vi "BSD_Filename Path formation_MS.vi"(6 "BF_name":string, 8 "error in (no error)":errorcluster caption="error in", 9 "Date":string, 10 "SAVE":bool=TRUE, 11 "Filename Path":path) -> (0 "error out":errorcluster, 1 "BNAL Path":T2, 2 "LS Path":T3, 3 "BS Path":T1, 4 "FN#":string)   [LabVIEW 2018]
panel:
  out "after substring":string
  out "after substring 4":string
  out "BS_S Path":string
  out "BS_J Path":string
  out "BS_CP Path":string
  out "B_TDMS Path":string
  out "B_Folder Path":string
  out "LSE Path":string
  out "BS_T Path":string
  out "LS Signal Table Path":path
  out "LS CP Table Path":path
  out "LS Time Table Path":path
  out "Ex Con":string
  out "B_TDMS F_Name":string
  out "B_Folder name":string
  out "Pre File F_Name":string
  out "File location folder":string
  out "B Signal Table Path":path
  out "B CP Table Path":path
  out "B Time Table Path":path
  out "Filename":string
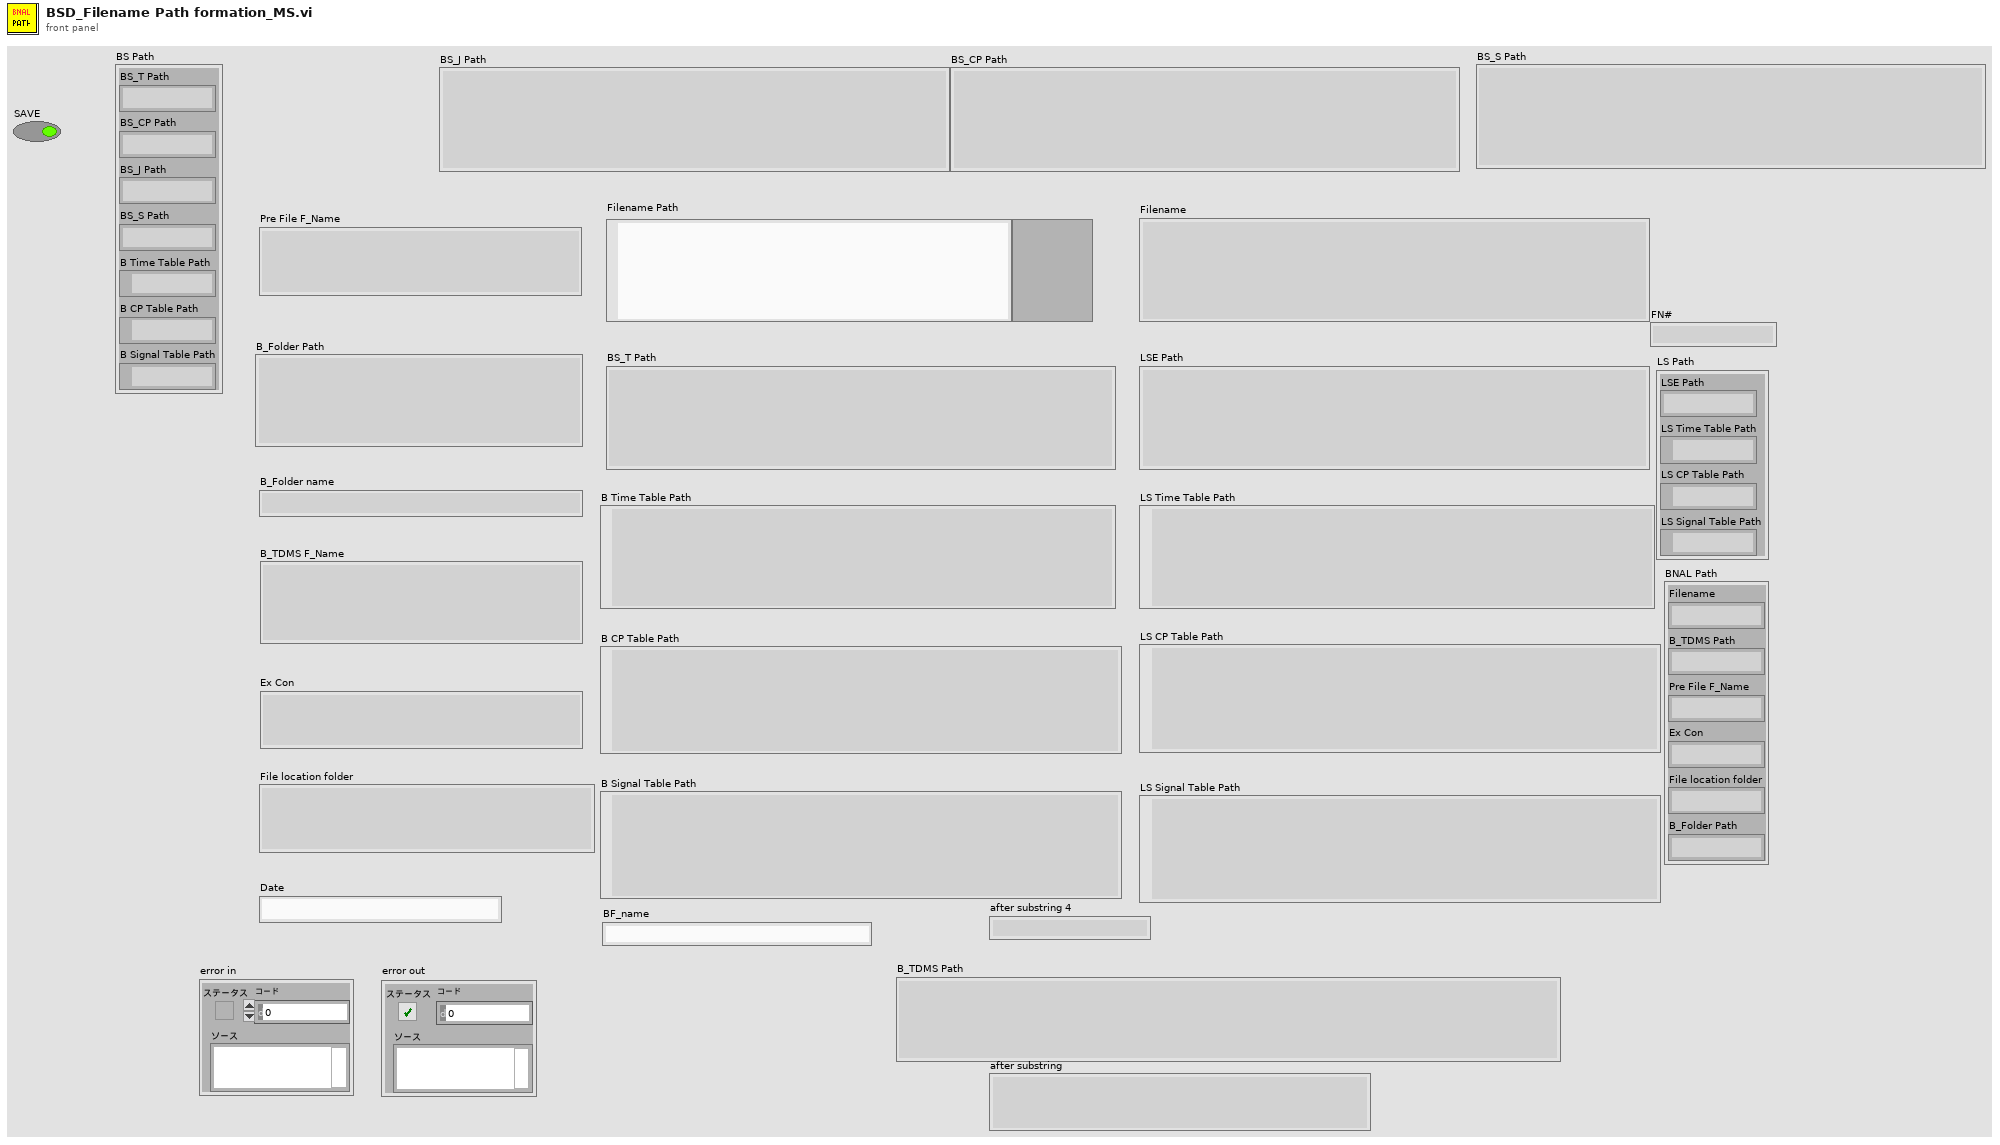
[diagram p1: front panel]
types:
  T1 = cluster{"BS_T Path":string, "BS_CP Path":string, "BS_J Path":string, "BS_S Path":string, "B Time Table Path":path, "B CP Table Path":path, "B Signal Table Path":path}
  T2 = cluster{"Filename":string, "B_TDMS Path":string, "Pre File F_Name":string, "Ex Con":string, "File location folder":string, "B_Folder Path":string}
  T3 = cluster{"LSE Path":string, "LS Time Table Path":path, "LS CP Table Path":path, "LS Signal Table Path":path}
  T4 = cluster{"name":string, string, string, string, string, string}
  T5 = cluster{string, string, string, string, path, path, path}
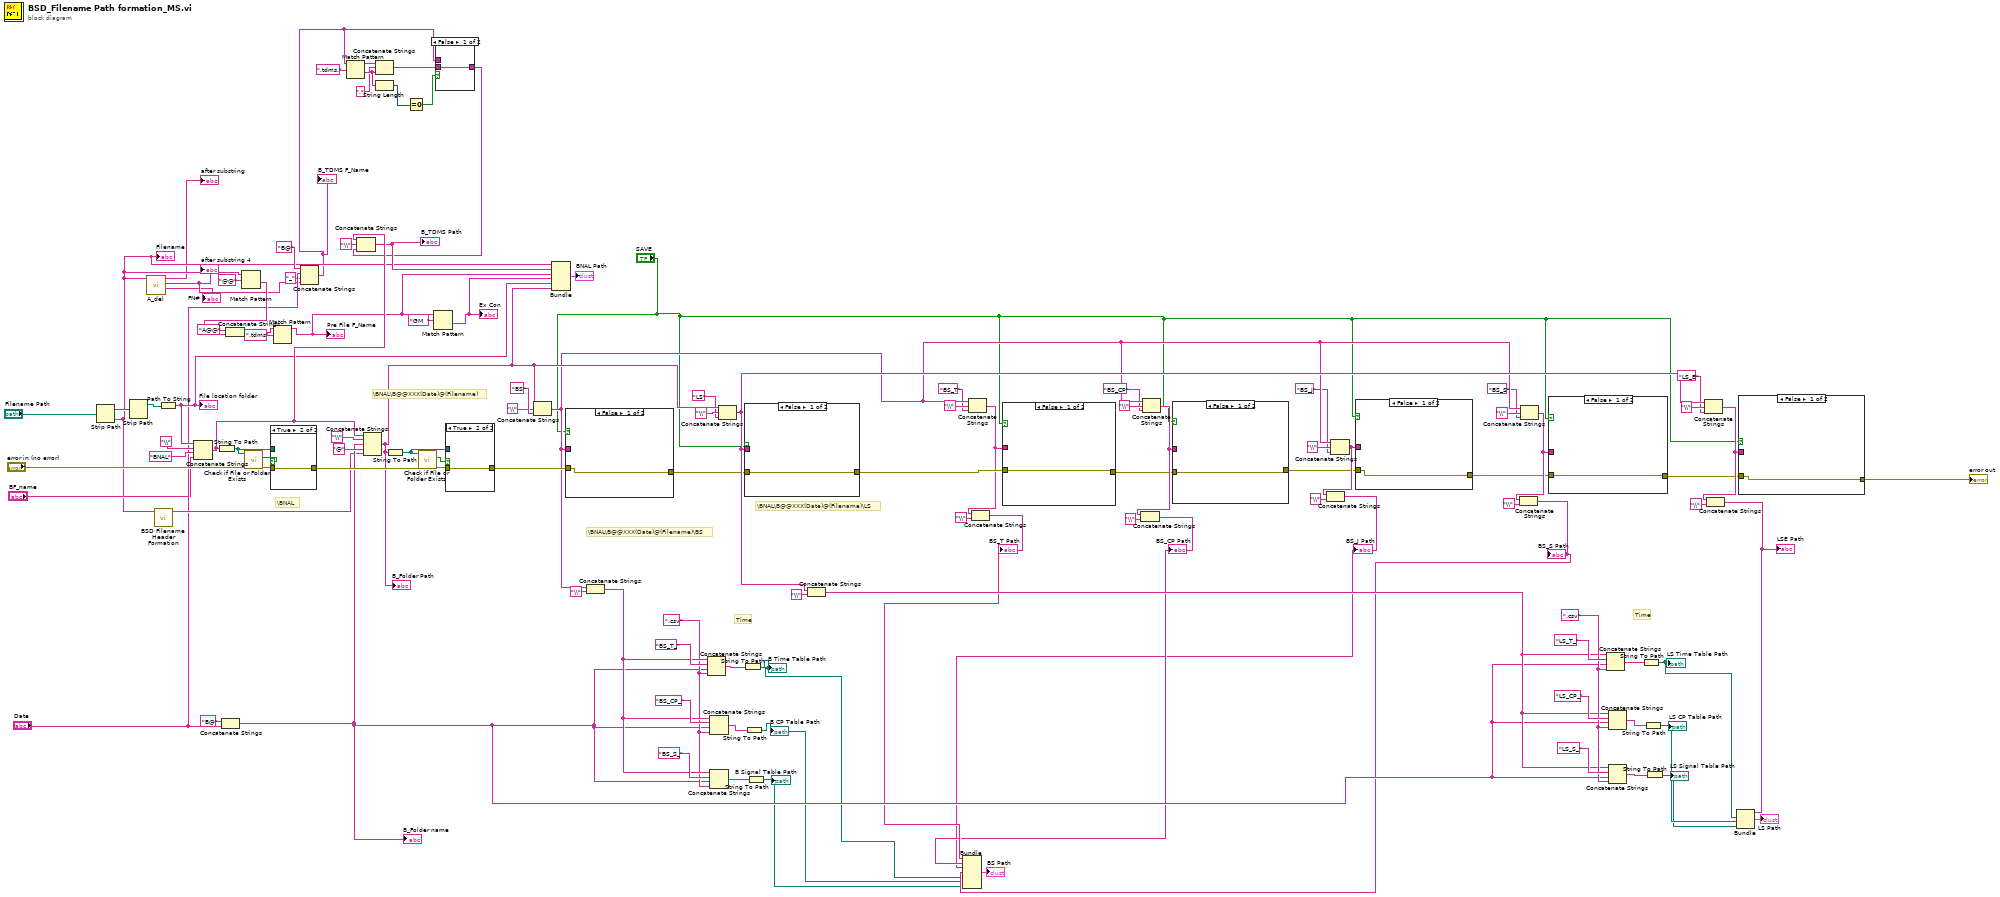
[diagram p0: block diagram]
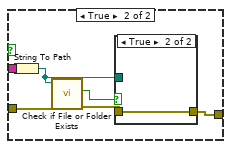
[diagram p3: hidden frame]
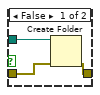
[diagram p4: hidden frame]
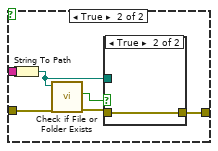
[diagram p5: hidden frame]
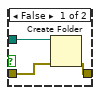
[diagram p6: hidden frame]
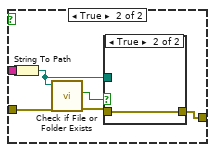
[diagram p7: hidden frame]
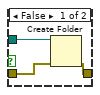
[diagram p8: hidden frame]
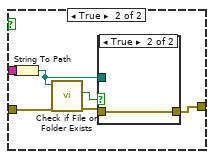
[diagram p9: hidden frame]
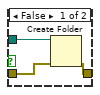
[diagram p10: hidden frame]
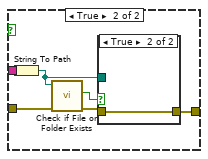
[diagram p11: hidden frame]
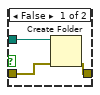
[diagram p12: hidden frame]
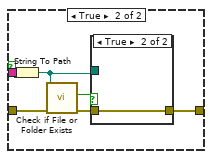
[diagram p13: hidden frame]
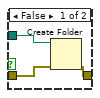
[diagram p14: hidden frame]
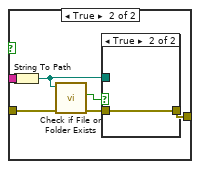
[diagram p15: hidden frame]
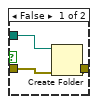
[diagram p16: hidden frame]
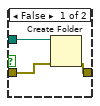
[diagram p17: hidden frame]
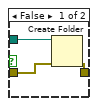
[diagram p18: hidden frame]
diagram:
  w78 = ".csv" ("文字列")
  w85 = ".csv" ("文字列")
  # "\\BNAL\\B@@XXX(Date)@(Filename)\\LS"
  # "\\BNAL\\B@@XXX(Date)@(Filename)\\BS"
  # "Time"
  # "\\BNAL\\B@@XXX(Date)@(Filename)"
  # "\\BNAL"
  # "Time"
  n1 = Strip Path(path="Filename Path") -> (stripped path=w68:path, name=w14:string)
  "Filename" <- w14
  n2 = Strip Path(path=w68) -> (stripped path=w87:path)  [unwired: 1 out]
  n3 = call "A_del.vi"("Filename"=w14) -> ("before substring 2"=→"FN#":string, "after substring 4"=w13:string, "after substring"=→"after substring":string)  [unwired: 8 in]
  "after substring 4" <- w13
  n4 = call "BSD Filename Header Formation.vi"("Pre File F_Name"=w14) -> ("Head for BNAL"=w49:string)  [unwired: 10 in]
  n5 = Path To String(path=w87) -> (string=w60:string)
  "File location folder" <- w60
  n6 = Concatenate Strings(w60, "\\" ("文字列"), "BNAL" ("文字列"), "BF_name") -> (w66:string)
  n7 = String To Path(string=w66) -> (path=w104:path)
  n8 = Concatenate Strings("B@" ("文字列"), "Date") -> (w76:string)
  "B_Folder name" <- w76
  n9 = Match Pattern(string=w14, regular expression="@@" ("正規表現")) -> (after substring=w50:string)  [unwired: 1 in, 3 out]
  n10 = Concatenate Strings("A@@" ("文字列"), w50) -> (w91:string)
  n11 = call <vilib>:"Check if File or Folder Exists.vi"("error in (no error)"="error in (no error)", "path"=w104) -> ("error out"=w102:errorcluster, "file or folder exists?"=w103:bool)  [unwired: 7 in, 1 out]
  n12 = case shown="True" w103 {
    tunnel: w104 -> [w118 _]
    tunnel: w102 -> [w117 w119]
    tunnel: [w116 w119] -> w95
    frame False {
      n13 = Create Folder(path (use dialog)=w118, error in=w117) -> (error out=w116:errorcluster)  [unwired: 1 in, 2 out]
    }
    frame True {
    }
  }
  n14 = Match Pattern(string=w91, regular expression=".tdms" ("正規表現")) -> (before substring=w63:string)  [unwired: 1 in, 3 out]
  "Pre File F_Name" <- w63
  n15 = Concatenate Strings("B@" ("文字列"), "Date", "_" ("string"), w13) -> (w2:string)
  "B_TDMS F_Name" <- w2
  n16 = Match Pattern(string=w2, regular expression=".tdms.") -> (before substring=w6:string, after substring=w5:string)  [unwired: 1 in, 2 out]
  n17 = Concatenate Strings(w66, "\\" ("文字列"), w76, "@" ("文字列"), w49) -> (w61:string)
  "B_Folder Path" <- w61
  n18 = Concatenate Strings(w6, "." ("string"), w5) -> (w3:string)
  n19 = String Length(string=w5) -> (length=w8:i32)
  n20 = String To Path(string=w61) -> (path=w98:path)
  n21 = Equal To 0?(x=w8) -> (x = 0?=w7:bool)
  n22 = call <vilib>:"Check if File or Folder Exists.vi"("error in (no error)"=w95, "path"=w98) -> ("error out"=w96:errorcluster, "file or folder exists?"=w97:bool)  [unwired: 7 in, 1 out]
  n23 = Match Pattern(string=w63, regular expression="GM  " ("正規表現")) -> (after substring=w62:string)  [unwired: 1 in, 3 out]
  "Ex Con" <- w62
  n24 = case shown="False" w7 {
    tunnel: w2 -> [_ w121]
    tunnel: [w120 w121] -> w1
    tunnel: w3 -> [w120 _]
    frame False {
    }
    frame True {
    }
  }
  n25 = Concatenate Strings(w66, "\\" ("文字列"), w1) -> (w64:string)
  "B_TDMS Path" <- w64
  n26 = case shown="True" w97 {
    tunnel: w98 -> [w124 _]
    tunnel: w96 -> [w123 w125]
    tunnel: [w122 w125] -> w94
    frame False {
      n27 = Create Folder(path (use dialog)=w124, error in=w123) -> (error out=w122:errorcluster)  [unwired: 1 in, 2 out]
    }
    frame True {
    }
  }
  n28 = Concatenate Strings(w61, "\\" ("文字列"), "BS" ("文字列")) -> (w51:string)
  n29 = Bundle("name"=w14, w64, w63, w62, w60, w61) -> (→"BNAL Path":T4)  [unwired: 1 in]
  n30 = case shown="False" "SAVE" {
    tunnel: w94 -> [w126 w132]
    tunnel: w51 -> [_ w131]
    tunnel: [w126 w127] -> w44
    frame False {
    }
    frame True {
      n31 = String To Path(string=w131) -> (path=w130:path)
      n32 = call <vilib>:"Check if File or Folder Exists.vi"("error in (no error)"=w132, "path"=w130) -> ("error out"=w128:errorcluster, "file or folder exists?"=w129:bool)  [unwired: 7 in, 1 out]
      n33 = case shown="True" w129 {
        tunnel: w130 -> [w135 _]
        tunnel: w128 -> [w134 w136]
        tunnel: [w133 w136] -> w127
        frame False {
          n34 = Create Folder(path (use dialog)=w135, error in=w134) -> (error out=w133:errorcluster)  [unwired: 1 in, 2 out]
        }
        frame True {
        }
      }
    }
  }
  n35 = Concatenate Strings(w51, "\\" ("文字列")) -> (w86:string)
  n36 = Concatenate Strings(w86, "BS_T_" ("文字列"), w76, w85) -> (w113:string)
  n37 = Concatenate Strings(w86, "BS_CP_" ("文字列"), w76, w85) -> (w112:string)
  n38 = Concatenate Strings(w86, "BS_S_" ("文字列"), w76, w85) -> (w111:string)
  n39 = Concatenate Strings(w61, "\\" ("文字列"), "LS" ("文字列")) -> (w75:string)
  n40 = String To Path(string=w113) -> (path=w54:path)
  "B Time Table Path" <- w54
  n41 = case shown="False" "SAVE" {
    tunnel: w75 -> [_ w143]
    tunnel: w44 -> [w137 w140]
    tunnel: [w137 w139] -> w43
    frame False {
    }
    frame True {
      n42 = String To Path(string=w143) -> (path=w138:path)
      n43 = call <vilib>:"Check if File or Folder Exists.vi"("error in (no error)"=w140, "path"=w138) -> ("error out"=w141:errorcluster, "file or folder exists?"=w142:bool)  [unwired: 7 in, 1 out]
      n44 = case shown="True" w142 {
        tunnel: w138 -> [w146 _]
        tunnel: w141 -> [w145 w147]
        tunnel: [w144 w147] -> w139
        frame False {
          n45 = Create Folder(path (use dialog)=w146, error in=w145) -> (error out=w144:errorcluster)  [unwired: 1 in, 2 out]
        }
        frame True {
        }
      }
    }
  }
  n46 = String To Path(string=w112) -> (path=w53:path)
  "B CP Table Path" <- w53
  n47 = String To Path(string=w111) -> (path=w52:path)
  "B Signal Table Path" <- w52
  n48 = Concatenate Strings(w75, "\\" ("文字列")) -> (w77:string)
  n49 = Concatenate Strings(w51, "\\" ("文字列"), "BS_T" ("文字列")) -> (w38:string)
  n50 = Concatenate Strings(w38, "\\" ("文字列")) -> (w58:string)
  "BS_T Path" <- w58
  n51 = case shown="False" "SAVE" {
    tunnel: w43 -> [w148 w152]
    tunnel: w38 -> [_ w150]
    tunnel: [w148 w149] -> w28
    frame False {
    }
    frame True {
      n52 = String To Path(string=w150) -> (path=w151:path)
      n53 = call <vilib>:"Check if File or Folder Exists.vi"("error in (no error)"=w152, "path"=w151) -> ("error out"=w153:errorcluster, "file or folder exists?"=w154:bool)  [unwired: 7 in, 1 out]
      n54 = case shown="True" w154 {
        tunnel: w151 -> [w157 _]
        tunnel: w153 -> [w156 w158]
        tunnel: [w155 w158] -> w149
        frame False {
          n55 = Create Folder(path (use dialog)=w157, error in=w156) -> (error out=w155:errorcluster)  [unwired: 1 in, 2 out]
        }
        frame True {
        }
      }
    }
  }
  n56 = Concatenate Strings(w51, "\\" ("文字列"), "BS_CP" ("文字列")) -> (w29:string)
  n57 = Concatenate Strings(w29, "\\" ("文字列")) -> (w57:string)
  "BS_CP Path" <- w57
  n58 = case shown="False" "SAVE" {
    tunnel: w29 -> [_ w162]
    tunnel: w28 -> [w159 w161]
    tunnel: [w159 w160] -> w24
    frame False {
    }
    frame True {
      n59 = String To Path(string=w162) -> (path=w163:path)
      n60 = call <vilib>:"Check if File or Folder Exists.vi"("error in (no error)"=w161, "path"=w163) -> ("error out"=w164:errorcluster, "file or folder exists?"=w165:bool)  [unwired: 7 in, 1 out]
      n61 = case shown="True" w165 {
        tunnel: w163 -> [w168 _]
        tunnel: w164 -> [w167 w169]
        tunnel: [w166 w169] -> w160
        frame False {
          n62 = Create Folder(path (use dialog)=w168, error in=w167) -> (error out=w166:errorcluster)  [unwired: 1 in, 2 out]
        }
        frame True {
        }
      }
    }
  }
  n63 = Concatenate Strings(w51, "\\" ("文字列"), "BS_J" ("文字列")) -> (w25:string)
  n64 = Concatenate Strings(w25, "\\" ("文字列")) -> (w56:string)
  "BS_J Path" <- w56
  n65 = case shown="False" "SAVE" {
    tunnel: w25 -> [_ w173]
    tunnel: w24 -> [w170 w172]
    tunnel: [w170 w171] -> w19
    frame False {
    }
    frame True {
      n66 = String To Path(string=w173) -> (path=w174:path)
      n67 = call <vilib>:"Check if File or Folder Exists.vi"("error in (no error)"=w172, "path"=w174) -> ("error out"=w175:errorcluster, "file or folder exists?"=w176:bool)  [unwired: 7 in, 1 out]
      n68 = case shown="True" w176 {
        tunnel: w174 -> [w179 _]
        tunnel: w175 -> [w178 w180]
        tunnel: [w177 w180] -> w171
        frame False {
          n69 = Create Folder(path (use dialog)=w179, error in=w178) -> (error out=w177:errorcluster)  [unwired: 1 in, 2 out]
        }
        frame True {
        }
      }
    }
  }
  n70 = Concatenate Strings(w51, "\\" ("文字列"), "BS_S" ("文字列")) -> (w20:string)
  n71 = Concatenate Strings(w20, "\\" ("文字列")) -> (w55:string)
  "BS_S Path" <- w55
  n72 = Bundle(w58, w57, w56, w55, w54, w53, w52) -> (→"BS Path":T5)  [unwired: 1 in]
  n73 = case shown="False" "SAVE" {
    tunnel: w20 -> [_ w184]
    tunnel: w19 -> [w181 w183]
    tunnel: [w181 w182] -> w18
    frame False {
    }
    frame True {
      n74 = String To Path(string=w184) -> (path=w185:path)
      n75 = call <vilib>:"Check if File or Folder Exists.vi"("error in (no error)"=w183, "path"=w185) -> ("error out"=w186:errorcluster, "file or folder exists?"=w187:bool)  [unwired: 7 in, 1 out]
      n76 = case shown="True" w187 {
        tunnel: w185 -> [w190 _]
        tunnel: w186 -> [w189 w191]
        tunnel: [w188 w191] -> w182
        frame False {
          n77 = Create Folder(path (use dialog)=w190, error in=w189) -> (error out=w188:errorcluster)  [unwired: 1 in, 2 out]
        }
        frame True {
        }
      }
    }
  }
  n78 = Concatenate Strings(w77, "LS_T_" ("文字列"), w76, w78) -> (w84:string)
  n79 = Concatenate Strings(w77, "LS_CP_" ("文字列"), w76, w78) -> (w83:string)
  n80 = Concatenate Strings(w77, "LS_S_" ("文字列"), w76, w78) -> (w82:string)
  n81 = String To Path(string=w84) -> (path=w71:path)
  "LS Time Table Path" <- w71
  n82 = String To Path(string=w83) -> (path=w70:path)
  "LS CP Table Path" <- w70
  n83 = String To Path(string=w82) -> (path=w69:path)
  "LS Signal Table Path" <- w69
  n84 = Concatenate Strings(w75, "\\" ("文字列"), "LS_E" ("文字列")) -> (w34:string)
  n85 = Concatenate Strings(w34, "\\" ("文字列")) -> (w72:string)
  "LSE Path" <- w72
  n86 = Bundle(w72, w71, w70, w69) -> (→"LS Path":cluster{string, path, path, path})  [unwired: 1 in]
  n87 = case shown="False" "SAVE" {
    tunnel: [w192 w198] -> w74
    tunnel: w34 -> [_ w194]
    tunnel: w18 -> [w192 w193]
    frame False {
    }
    frame True {
      n88 = String To Path(string=w194) -> (path=w195:path)
      n89 = call <vilib>:"Check if File or Folder Exists.vi"("error in (no error)"=w193, "path"=w195) -> ("error out"=w196:errorcluster, "file or folder exists?"=w197:bool)  [unwired: 7 in, 1 out]
      n90 = case shown="True" w197 {
        tunnel: w195 -> [w201 _]
        tunnel: w196 -> [w200 w202]
        tunnel: [w199 w202] -> w198
        frame False {
          n91 = Create Folder(path (use dialog)=w201, error in=w200) -> (error out=w199:errorcluster)  [unwired: 1 in, 2 out]
        }
        frame True {
        }
      }
    }
  }
  "error out" <- w74
